vi "example test.vi"() -> (0 "final error":errorcluster)   [LabVIEW 2013, in "CVT tests.lvlib"]
uses:
  CVT tests.lvlib
  execution/CVT runtime.lvclass
  configuration/CVT configuration.lvclass
  <vilib>/NI/Tag Bus/tag/Data Type.ctl
  <vilib>/NI/Tag Bus Module Framework/channel/channel classification.ctl
  <vilib>/NI/Tag Bus/dictionary/data dictionary.lvclass/data dictionary.ctl
  <vilib>/NI/Tag Bus/dictionary/lookup polymorphs/locate double.vi
  <vilib>/NI/Tag Bus/table/data polymorphs/write one/write Double.vi
  <vilib>/NI/Tag Bus/table/data polymorphs/read one/read Double.vi
  <vilib>/NI/Tag Bus/dictionary/search/find data index.vi
  <vilib>/NI/Tag Bus/dictionary/search/search string list.vi
  <vilib>/NI/Tag Bus/dictionary/tag not found.vi
  <vilib>/NI/Tag Bus Module Framework/channel/TBM channel.lvclass
  <vilib>/NI/Tag Bus/tag/tag descriptor.lvclass
  <vilib>/NI/Tag Bus/dictionary/data dictionary.lvclass
  <vilib>/NI/Tag Bus/table/data table.lvlib
  <vilib>/NI/Configuration Framework/serializable configuration/NISE_CEF_serializable configuration.lvclass
panel:
  in  "ch count":i32=100
  in  "for loop":i32=10000
  out "out usec/call":dbl
  out "in usec/call":dbl
  out "output error":errorcluster
  out "input error":errorcluster
  out "output lookup error":errorcluster
  out "no data written":bool
  out "input lookup error":errorcluster
  out "init error":errorcluster
  out "correct execution settings":bool
  out "serialization problem":errorcluster
  out "invalid configuration":errorcluster
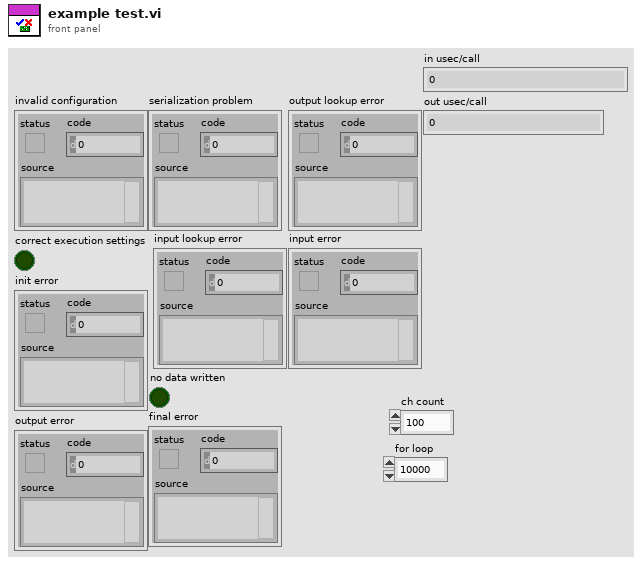
[diagram p1: front panel]
types:
  T1 = typedef "TBM channel.lvclass/channel classification.ctl" = enum16{"input data", "output data", "processing parameter", "processing result"}
  T2 = typedef "tag bus.lvlib/tag descriptor.lvclass/Data Type.ctl" = enum16{"Double", "Single", "I64", "I32", "I16", "I8", "U64", "U32", "U16", "U8", "Boolean", "String", "Array of Double", "Array of Single", "Array of I64", "Array of I32", "Array of I16", "Array of I8", "Array of U64", "Array of U32", "Array of U16", "Array of U8", "Array of Boolean", "Array of String"}
  T3 = typedef "TBM channel.lvclass/data tables.ctl" = cluster{"input data":T4, "processing parameter":T4, "processing result":T4, "output data":T4}
  T4 = typedef "tag bus.lvlib/dictionary table pair.ctl" = cluster{"data dictionary":refnum<class "data dictionary.lvclass">, "data table":T5}
  T5 = typedef "tag bus.lvlib/data table.lvlib/data table.ctl" = cluster{"Double":dbl[], "Single":sgl[], "I64":i64[], "I32":i32[], "I16":i16[], "I8":i8[], "U64":u64[], "U32":u32[], "U16":u16[], "U8":u8[], "Boolean":bool[], "String":string[], "Array of Double":cluster{"DBL Array":dbl[]}[], "Array of Single":cluster{"SGL Array":sgl[]}[], "Array of I64":cluster{"I64 Array":i64[]}[], "Array of I32":cluster{"I32 Array":i32[]}[], "Array of I16":cluster{"I16 Array":i16[]}[], "Array of I8":cluster{"I8 Array":i8[]}[], "Array of U64":cluster{"U64 Array":u64[]}[], "Array of U32":cluster{"U32 Array":u32[]}[], "Array of U16":cluster{"U16 Array":u16[]}[], "Array of U8":cluster{"U8 Array":u8[]}[], "Array of Boolean":cluster{"Boolean Array":bool[]}[], "Array of String":cluster{"String Array":string[]}[]}
  T6 = typedef "TBM module execution interface.lvclass/execution settings.ctl" = cluster{"reads inputs":bool, "processes data":bool, "writes outputs":bool}
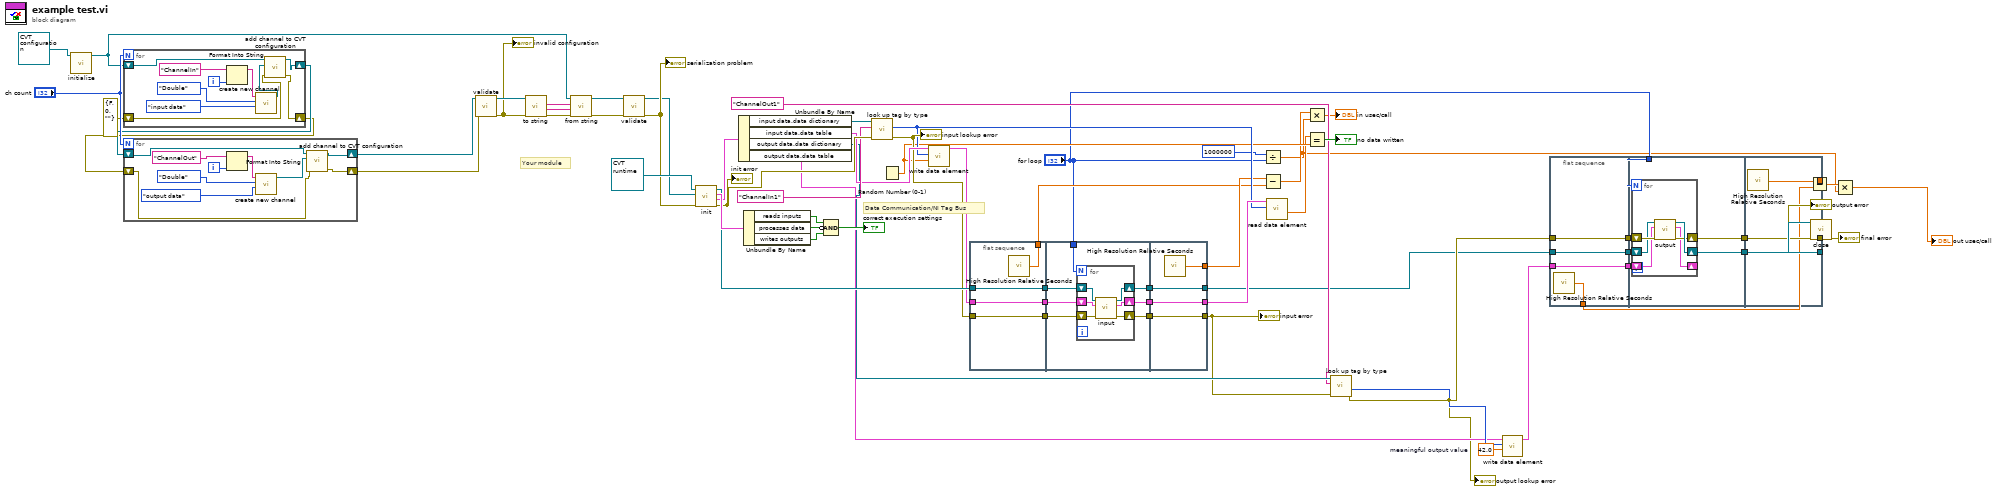
[diagram p0: block diagram]
diagram:
  w37 = 42.0  # meaningful output value
  # "Data Communication/NI Tag Bus"
  # "Your module"
  n1 = call <vilib>:"initialize.vi"("configuration in"=refnum<class "CVT configuration.lvclass"> refnum ("tag bus configurable plugin module configuration")) -> ("configuration out"=w1:refnum<class "CVT configuration.lvclass">)  [unwired: 8 in, 2 out]
  n2 = for {
    N: "ch count" -> [_]
    shift-right: [w74] -> w7
    shift-left: w1 -> [w73]
    shift-right: [w75] -> w4
    shift-left: errorcluster {"status"=FALSE, "code"=0, "source"=""} ("error out") -> [w71]
    i -> [w78]
    n3 = Format Into String(initial string="ChannelIn" ("channel name"), w78) -> (resulting string=w77:string)  [unwired: 2 in, 1 out]
    n4 = call <vilib>:"create new channel.vi"("channel classification"=channel_classification."input data", "data type"=Data_Type."Double", "channel name"=w77) -> ("channel"=w72:refnum<class "TBM channel.lvclass">)  [unwired: 8 in]
    n5 = call "add channel to CVT configuration.vi"("error in"=w71, "channel"=w72, "CVT configuration in"=w73) -> ("error out"=w75:errorcluster, "CVT configuration out"=w74:refnum<class "CVT configuration.lvclass">)  [unwired: 7 in]
  }
  n6 = for {
    N: "ch count" -> [_]
    shift-right: [w82] -> w6
    shift-left: w7 -> [w85]
    shift-right: [w83] -> w5
    shift-left: w4 -> [w84]
    i -> [w88]
    n7 = Format Into String(initial string="ChannelOut" ("channel name"), w88) -> (resulting string=w87:string)  [unwired: 2 in, 1 out]
    n8 = call <vilib>:"create new channel.vi"("channel classification"=channel_classification."output data", "data type"=Data_Type."Double", "channel name"=w87) -> ("channel"=w81:refnum<class "TBM channel.lvclass">)  [unwired: 8 in]
    n9 = call "add channel to CVT configuration.vi"("error in"=w84, "channel"=w81, "CVT configuration in"=w85) -> ("error out"=w83:errorcluster, "CVT configuration out"=w82:refnum<class "CVT configuration.lvclass">)  [unwired: 7 in]
  }
  n10 = call-dynamic "validate.vi"("error in"=w5, "CVT configuration in"=w6) -> ("error out"=w69:errorcluster, "CVT configuration out"=w70:refnum<class "CVT configuration.lvclass">)  [unwired: 8 in]
  "invalid configuration" <- w69
  n11 = call-dynamic "to string.vi"("error in"=w69, "CVT configuration in"=w70) -> ("error out"=w66:errorcluster, "data"=w67:string, "version"=w68:string)  [unwired: 6 in, 1 out]
  n12 = call-dynamic "from string.vi"("error in"=w66, "data"=w67, "version"=w68, "CVT configuration in"=w1) -> ("error out"=w64:errorcluster, "CVT configuration out"=w65:refnum<class "CVT configuration.lvclass">)  [unwired: 6 in]
  n13 = call-dynamic "validate.vi"("error in"=w64, "CVT configuration in"=w65) -> ("error out"=w62:errorcluster, "CVT configuration out"=w61:refnum<class "CVT configuration.lvclass">)  [unwired: 8 in]
  "serialization problem" <- w62
  n14 = call-dynamic "init.vi"("error in"=w62, "TBM module configuration in"=w61, "CVT runtime in"=refnum<class "CVT runtime.lvclass"> refnum ("tag bus configurable plugin module")) -> ("error out"=w53:errorcluster, "data allocations"=w55:T3, "execution settings"=w60:T6, "CVT runtime out"=w50:refnum<class "CVT runtime.lvclass">)  [unwired: 5 in]
  "init error" <- w53
  n15 = Unbundle By Name(w55) -> ("input data.data dictionary"=w54:refnum<class "data dictionary.lvclass">, "input data.data table"=w51:T5, "output data.data dictionary"=w42:refnum<class "data dictionary.lvclass">, "output data.data table"=w39:T5)
  n16 = Unbundle By Name(w60) -> ("reads inputs"=w57:bool, "processes data"=w59:bool, "writes outputs"=w58:bool)
  n17 = Compound Arithmetic op=AND(w57, invert w59, w58) -> (→"correct execution settings":bool)
  n18 = call-poly <vilib>:"look up tag by type.vi"("error in"=w53, "name"="ChannelIn1" ("channel name"), "data dictionary in"=w54) -> ("error out"=w49:errorcluster, "index"=w46:i32)  [unwired: 6 in, 1 out]
  "input lookup error" <- w49
  n19 = Random Number (0-1)() -> (number: 0 to 1=w45:dbl)
  n20 = call-poly <vilib>:"write data element.vi"("value"=w45, "index"=w46, "data table in"=w51) -> ("data table out"=w48:T5)  [unwired: 8 in]
  n21 = flat-sequence {
    tunnel: w48 -> [w92]
    tunnel: w49 -> [w93]
    tunnel: w50 -> [w94]
    tunnel: [w94] -> w27
    tunnel: [w93] -> w26
    tunnel: [w92] -> w25
    tunnel: [w91] -> w23
    tunnel: [w98] -> w30
    tunnel: [w97] -> w29
    tunnel: [w96] -> w28
    tunnel: w27 -> [w101]
    tunnel: w26 -> [w100]
    tunnel: w25 -> [w99]
    tunnel: "for loop" -> [w95]
    tunnel: [w109] -> w35
    tunnel: [w110] -> w38
    tunnel: [w111] -> w47
    tunnel: w30 -> [w111]
    tunnel: w29 -> [w110]
    tunnel: w28 -> [w109]
    tunnel: [w108] -> w24
    frame #0 {
      n22 = call <vilib>:"High Resolution Relative Seconds.vi"() -> ("relative seconds"=w91:dbl)
    }
    frame #1 {
      n23 = for {
        N: w95 -> [_]
        shift-right: [w102] -> w96
        shift-left: w101 -> [w107]
        shift-right: [w104] -> w98
        shift-left: w99 -> [w105]
        shift-right: [w103] -> w97
        shift-left: w100 -> [w106]
        n24 = call-dynamic "input.vi"("error in"=w106, "data table in"=w105, "CVT runtime in"=w107) -> ("error out"=w103:errorcluster, "data table out"=w104:T5, "CVT runtime out"=w102:refnum<class "CVT runtime.lvclass">)  [unwired: 6 in]
      }
    }
    frame #2 {
      n25 = call <vilib>:"High Resolution Relative Seconds.vi"() -> ("relative seconds"=w108:dbl)
    }
  }
  n26 = Divide(x=1000000, y="for loop") -> (x/y=w10:dbl)
  n27 = Subtract(x=w24, y=w23) -> (x-y=w13:dbl)
  n28 = call-poly <vilib>:"read data element.vi"("index"=w46, "data table in"=w47) -> ("value"=w44:dbl)  [unwired: 8 in, 1 out]
  n29 = Multiply(x=w13, y=w10) -> (x*y=→"in usec/call":dbl)
  n30 = Equal?(x=w44, y=w45) -> (x = y?=→"no data written":bool)
  n31 = call-poly <vilib>:"look up tag by type.vi"("error in"=w38, "name"="ChannelOut1" ("channel name"), "data dictionary in"=w42) -> ("error out"=w36:errorcluster, "index"=w40:i32)  [unwired: 6 in, 1 out]
  "output lookup error" <- w36
  n32 = call-poly <vilib>:"write data element.vi"("value"=w37, "index"=w40, "data table in"=w39) -> ("data table out"=w34:T5)  [unwired: 8 in]
  n33 = flat-sequence {
    tunnel: w34 -> [w113]
    tunnel: w35 -> [w114]
    tunnel: w36 -> [w115]
    tunnel: [w115] -> w20
    tunnel: [w114] -> w19
    tunnel: [w113] -> w18
    tunnel: [w112] -> w16
    tunnel: [w118] -> w22
    tunnel: [w117] -> w21
    tunnel: w20 -> [w121]
    tunnel: w19 -> [w120]
    tunnel: w18 -> [w119]
    tunnel: "for loop" -> [w116]
    tunnel: [w129] -> w32
    tunnel: [w130] -> w33
    tunnel: w22 -> [w130]
    tunnel: w21 -> [w129]
    tunnel: [w128] -> w17
    frame #0 {
      n34 = call <vilib>:"High Resolution Relative Seconds.vi"() -> ("relative seconds"=w112:dbl)
    }
    frame #1 {
      n35 = for {
        N: w116 -> [_]
        shift-right: [w124] -> w118
        shift-left: w120 -> [w126]
        shift-right: [w123] -> w117
        shift-left: w121 -> [w127]
        shift-right: [w122] -> _
        shift-left: w119 -> [w125]
        n36 = call-dynamic "output.vi"("error in"=w127, "data table in"=w125, "CVT runtime in"=w126) -> ("error out"=w123:errorcluster, "data table out"=w122:T5, "CVT runtime out"=w124:refnum<class "CVT runtime.lvclass">)  [unwired: 6 in]
      }
    }
    frame #2 {
      n37 = call <vilib>:"High Resolution Relative Seconds.vi"() -> ("relative seconds"=w128:dbl)
    }
  }
  n38 = Subtract(x=w17, y=w16) -> (x-y=w11:dbl)
  n39 = call-dynamic "close.vi"("error in"=w32, "CVT runtime in"=w33) -> ("error out"=→"final error":errorcluster)  [unwired: 9 in]
  n40 = Multiply(x=w11, y=w10) -> (x*y=→"out usec/call":dbl)
  "input error" <- w38
  "output error" <- w32
